vi "Create Specific.vi"(7 "Direction":T2, 8 "error in (no error)":errorcluster, 9 "Topic Name":T1, 10 "Blackboard Reference":T3 {"refnum" format="%.0x"}, 11 "CIF_Iceoryx_BB in":refnum<class "CIF_Iceoryx_BB.lvclass">) -> (0 "error out":errorcluster, 1 "Data Variant":variant, 2 "Writer Reference":T4 {"refnum" format="%.0x"}, 3 "CIF_Iceoryx_BB out":refnum<class "CIF_Iceoryx_BB.lvclass">, 4 "Cluster or Array String":string)   [LabVIEW 2021, in "CIF_Iceoryx_BB.lvclass"]
uses:
  CIF_Iceoryx_BB.lvclass
  <vilib>/CIF Foundation/CIF Iceoryx/Refnum/Typedef/BB Writer Refnum.ctl
  <vilib>/CIF Foundation/CIF Iceoryx/Refnum/Typedef/BB Refnum.ctl
  ChannelCommon/typedef/Direction.ctl
  <vilib>/CIF Foundation/CIF Iceoryx/typedef/Topic Full Names.ctl
  CIF_Iceoryx_Chan/Typedef/Iceoryx Channel Error.ctl
  CIF_Iceoryx_Chan/SubVIs/Iceoryx Channel Errors Core.vi
  CIF_Iceoryx_Chan/CIF_Iceoryx_Chn.lvclass
  <vilib>/CIF Foundation/CIF Iceoryx/Iceoryx.lvlib
  ChannelCommon/ChannelCommon.lvlib
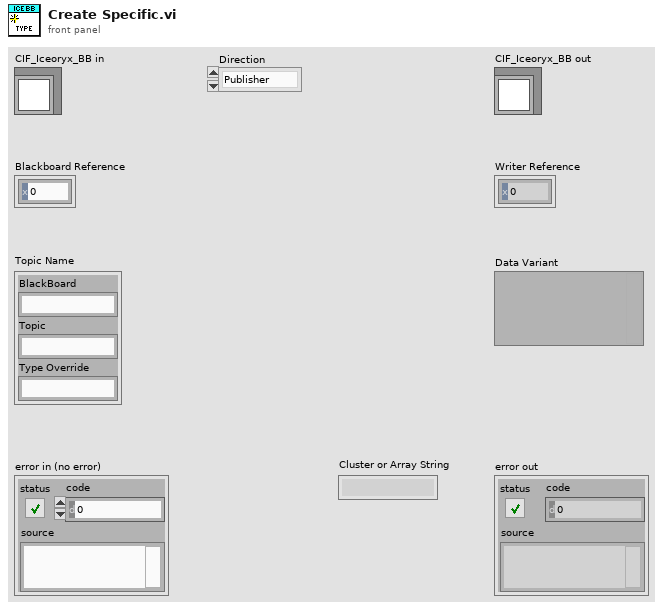
[diagram p1: front panel]
types:
  T1 = typedef "Iceoryx.lvlib/Topic Full Names.ctl" = cluster{"BlackBoard":string, "Topic":string, "Type Override":string}
  T2 = typedef "ChannelCommon.lvlib/Direction.ctl" = enum8{"Publisher", "Subscriber"}
  T3 = typedef "Iceoryx.lvlib/BB Refnum.ctl" = cluster{"refnum":u64, "BB":enum8{"bb"}}
  T4 = typedef "Iceoryx.lvlib/BB Writer Refnum.ctl" = cluster{"refnum":u64, "BB Writer":enum8{"bb_writer"}}
  T5 = typedef "CIF_Iceoryx_Chn.lvclass/Iceoryx Channel Error.ctl" = enum16{"Type Mismatch", "Name Mismatch", "Override Required"}
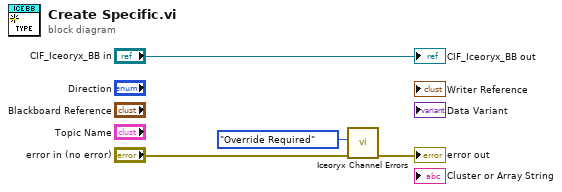
[diagram p0: block diagram]
diagram:
  n1 = call "Iceoryx Channel Errors.vi"("error in (no error)"="error in (no error)", "Error"=Iceoryx_Channel_Error."Override Required") -> ("error out"=→"error out":errorcluster)  [unwired: 9 in]
  "CIF_Iceoryx_BB out" <- "CIF_Iceoryx_BB in"
